vi "Get Signal Status.vi"(6 "ptrStopCount":u32, 7 "ptrStartCount":u32, 8 "error in (no error)":errorcluster caption="错误输入（无错误）", 9 "nChannel":i32, 10 "nBoard":i32, 11 "nDevId":i32) -> (0 "error out":errorcluster caption="错误输出", 3 "function return":i32, 4 "ptrStopCount out":u32, 5 "ptrStartCount out":u32)   [LabVIEW 2017, in "smncsftmt.lvlib"]
doc: "__declspec(dllexport) int GetSignalStatus(int nDevId, int nBoard, int nChannel, unsigned int* ptrStartCount, unsigned int* ptrStopCount);"
uses:
  smncsftmt.lvlib
  smncsftmt.dll
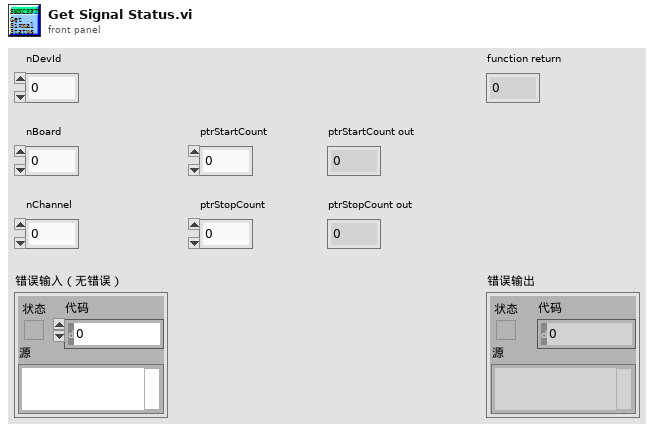
[diagram p1: front panel]
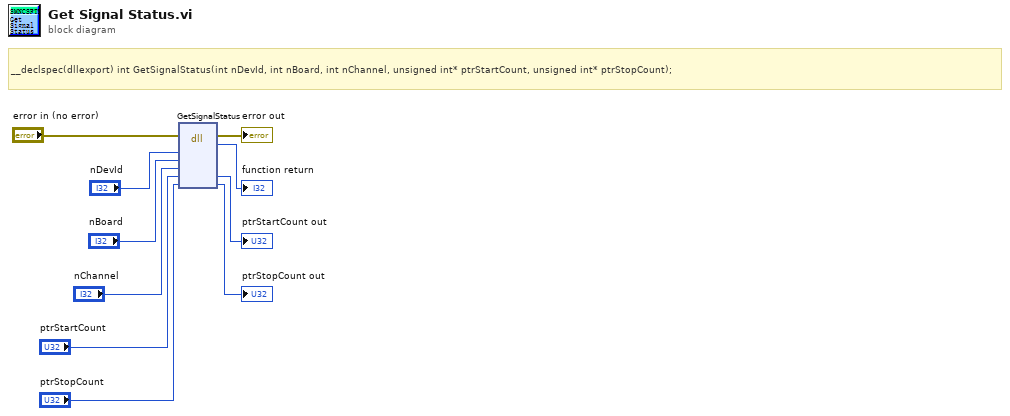
[diagram p0: block diagram]
diagram:
  # "__declspec(dllexport) int GetSignalStatus(int nDevId, int nBoard, int nChannel, unsigned int* ptrStartCount, unsigned int* ptrStopCount);"
  n1 = dll-call lib="PTH2oabs CUsersaDesktop\nLABVIEW范例National InstrumentsLabVIEW 2017user.lib\tsmncsftmtsmncsftmt.*" fn="GetSignalStatus"(error in="error in (no error)", "nDevId"="nDevId", "nBoard"="nBoard", "nChannel"="nChannel", "ptrStartCount"="ptrStartCount", "ptrStopCount"="ptrStopCount") -> (error out=→"error out":errorcluster, "返回类型"=→"function return":i32, "ptrStartCount"=→"ptrStartCount out":u32, "ptrStopCount"=→"ptrStopCount out":u32)  [unwired: 5 in, 1 out]
